vi "draw.vi"(0 "reference":refnum<class "FinalStateNode.lvclass">, 1 "graphics":refnum<class "Graphics.lvclass">, 5 "error in (no error)":errorcluster) -> (14 "reference out":refnum<class "FinalStateNode.lvclass">, 19 "error out":errorcluster)   [LabVIEW 2020, in "FinalStateNode.lvclass"]
doc: "public void draw(Graphics2D g2, Point2D p, Point2D q)"
uses:
  <resource>/Framework/Providers/Open_GDS/UML/FinalStateNode_class/FinalStateNode.lvclass
  C:/Program Files (x86)/National Instruments/LabVIEW 2020/resource/Framework/Providers/Open_GDS/UML/RectangularNode_class/RectangularNode.lvclass
  <resource>/Framework/Providers/Open_GDS/UML/Graphics_class/Graphics.lvclass
  <resource>/Framework/Providers/Open_GDS/UML/MultiLineString_class/MultiLineString.lvclass
  <resource>/Framework/Providers/Open_GDS/UML/RectangularNode_class/RectangularNode.lvclass
panel:
  in  "Case Constant\n(See Context Help)":bool
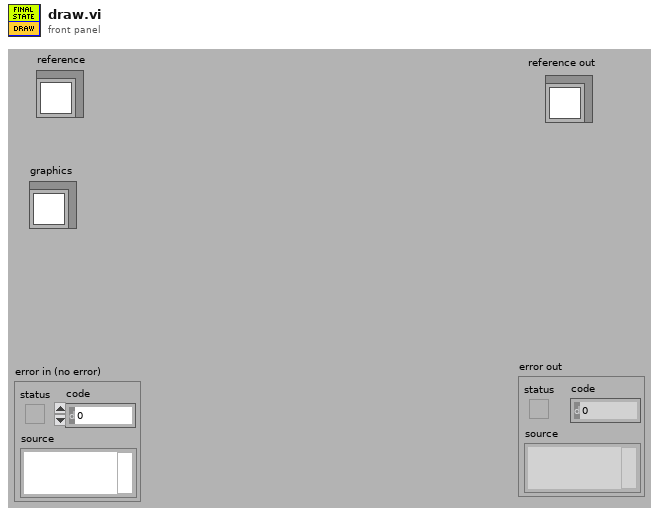
[diagram p1: front panel]
types:
  T1 = typedef "FinalStateNode.lvclass/ObjectAttributes.ctl" = cluster{"name":refnum<class "MultiLineString.lvclass">, "DEFAULT_WIDTH":i32, "DEFAULT_HEIGHT":i32}
  T2 = typedef "RectangularNode.lvclass/ObjectAttributes.ctl" = cluster{"bounds":T3}
  T3 = typedef "Rectangle Rectangle2D.ctl" = cluster{"x":dbl, "y":dbl, "width":dbl, "height":dbl}
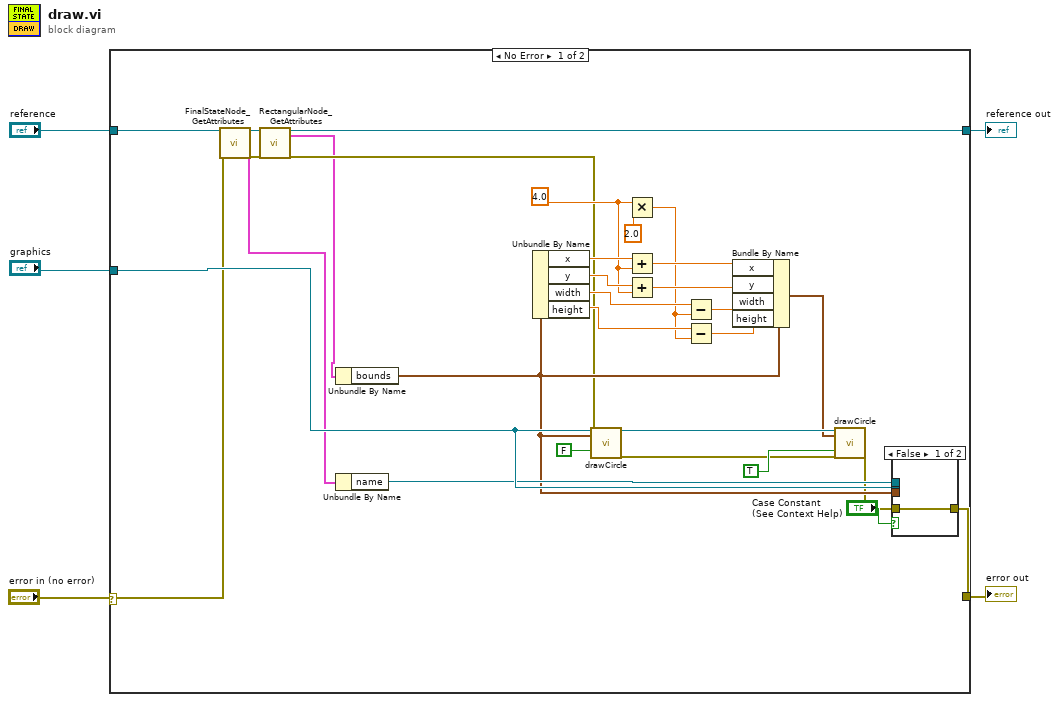
[diagram p0: block diagram]
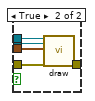
[diagram p2: hidden frame]
diagram:
  n1 = case shown="No Error" "error in (no error)" {
    selector: "error in (no error)" -> [w31 w42]
    tunnel: "reference" -> [w35 w43]
    tunnel: [w34 w42] -> w4
    tunnel: [w7 w43] -> w3
    tunnel: "graphics" -> [w33 _]
    frame No Error {
      w21 = 4.0
      n2 = call <resource>:"FinalStateNode_GetAttributes.vi"("reference in"=w35, "error in (no error)"=w31) -> ("reference out"=w10:refnum<class "FinalStateNode.lvclass">, "Data"=w11:T1, "error out"=w9:errorcluster)  [unwired: 1 in, 14 out]
      n3 = call <resource>:"RectangularNode_GetAttributes.vi"("reference in"=w10, "error in (no error)"=w9) -> ("reference out"=w7:refnum<class "FinalStateNode.lvclass">, "Data"=w6:T2, "error out"=w8:errorcluster)  [unwired: 14 in, 1 out]
      n4 = Unbundle By Name(w6) -> ("bounds"=w20:T3)
      n5 = Unbundle By Name(w11) -> ("name"=w32:refnum<class "MultiLineString.lvclass">)
      n6 = Unbundle By Name(w20) -> ("x"=w26:dbl, "y"=w25:dbl, "width"=w24:dbl, "height"=w23:dbl)
      n7 = call-dynamic "drawCircle.vi"("reference"=w33, "rectangle"=w20, "fill?(F)"=FALSE, "error in (no error)"=w8) -> ("reference out"=w28:refnum<class "Graphics.lvclass">, "error out"=w13:errorcluster)  [unwired: 14 in]
      n8 = Multiply(x=w21, y=2.0) -> (x*y=w15:dbl)
      n9 = Add(x=w26, y=w21) -> (x+y=w19:dbl)
      n10 = Add(x=w25, y=w21) -> (x+y=w18:dbl)
      n11 = Subtract(x=w24, y=w15) -> (x-y=w17:dbl)
      n12 = Subtract(x=w23, y=w15) -> (x-y=w16:dbl)
      n13 = Bundle By Name(cluster=w20, "x"=w19, "y"=w18, "width"=w17, "height"=w16) -> (w14:T3)
      n14 = call-dynamic "drawCircle.vi"("reference"=w28, "rectangle"=w14, "fill?(F)"=TRUE, "error in (no error)"=w13) -> ("error out"=w12:errorcluster)  [unwired: 14 in, 1 out]
      n15 = case shown="False" "Case Constant\n(See Context Help)" {
        tunnel: [w36 w41] -> w34
        tunnel: w33 -> [_ w40]
        tunnel: w32 -> [_ w39]
        tunnel: w12 -> [w36 w38]
        tunnel: w20 -> [_ w37]
        frame False {
        }
        frame True {
          n16 = call-dynamic "draw.vi"("reference"=w39, "graphics"=w40, "bounds"=w37, "error in (no error)"=w38) -> ("error out"=w41:errorcluster)  [unwired: 14 in, 1 out]
        }
      }
    }
    frame Error {
    }
  }
  "reference out" <- w3
  "error out" <- w4
